vi "Replace Tag with Array.vi"(8 "Error In":errorcluster caption="Error in (no error)", 9 "Tag":enum16{"<1>", "<2>", "<3>", "<4>"}(ring), 10 "Replace String":string[](array[string]), 11 "Single-line Text":string="All Data Saved@TDMS >> API: Terminate@<1> -><register>") -> (0 "Error Out":errorcluster, 3 "States":string)   [LabVIEW 2017, in "Communicable State Machine.lvlib"]
doc: "This VI is obsolete. Please use `CSM - Replace Mark with String Array.vi`\n\n### CSM - Replace Mark with String Array.vi\nReplaces tags in a single state string with strings from an array and merges them into a string describing a group of states.\n\n<b>Example</b>: For `Draw >> <1> -@ Painter`, <b>Tag</b> should be set to `<1>`\n\nInput array `[Line, Circle, Rectangle]`. The result will be:\n\n Draw >> Line -@ Painter\n Draw >> Circle -@ Painter\n Draw >> Rectangle -@ Painter\n\n-- <b>Controls</b> --\n- <b>single-line text</b>: Single-line state string containing tags like `<1>`, `<2>`, `<3>`, etc.\n- <b>Substitution Mark</b>: The tag to replace, such as `<1>`, `<2>`, `<3>`, etc.\n- <b>replace string</b>: The array of strings to replace the tag with.\n\n-- <b>Indicators</b> --\n- <b>States</b>: The merged state string."
uses:
  Communicable State Machine.lvlib
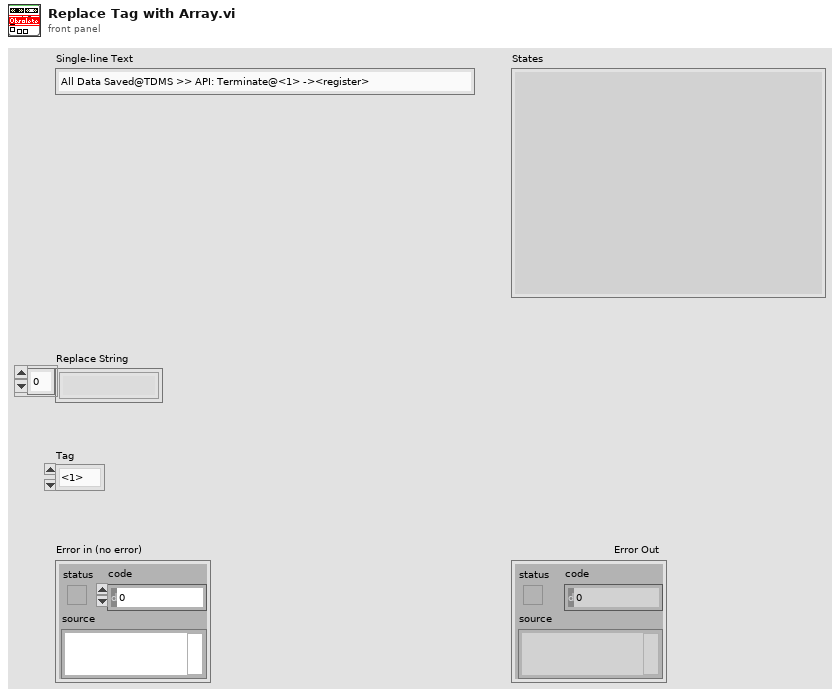
[diagram p1: front panel]
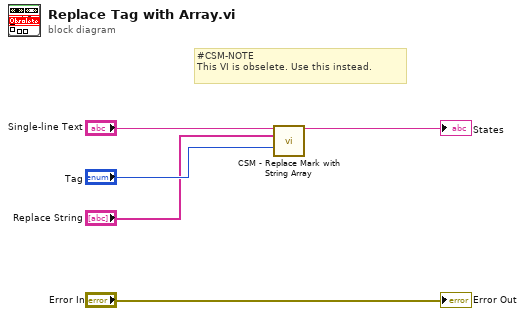
[diagram p0: block diagram]
diagram:
  # "#CSM-NOTE\nThis VI is obselete. Use this instead."
  n1 = call "CSM - Replace Mark with String Array.vi"("Single-line Text"="Single-line Text", "Replace String"="Replace String", "Substitution Mark"="Tag") -> ("States"=→"States":string)  [unwired: 12 in]
  "Error Out" <- "Error In"
